vi "getSerializedData.vi"(0 "reference":refnum<class "InterfaceNode.lvclass">, 5 "error in (no error)":errorcluster) -> (14 "reference out":refnum<class "InterfaceNode.lvclass">, 15 "parent":refnum<class "AbstractNode.lvclass">, 16 "children":refnum<class "AbstractNode.lvclass">[](array[class]), 17 "xmlOut":string, 19 "error out":errorcluster)   [LabVIEW 2020, in "InterfaceNode.lvclass"]
doc: "getSerializedData"
uses:
  <resource>/Framework/Providers/Open_GDS/UML/InterfaceNode_class/InterfaceNode.lvclass
  C:/Program Files (x86)/National Instruments/LabVIEW 2020/resource/Framework/Providers/Open_GDS/UML/ClassNode_class/ClassNode.lvclass
  C:/Program Files (x86)/National Instruments/LabVIEW 2020/resource/Framework/Providers/Open_GDS/UML/RectangularNode_class/RectangularNode.lvclass
  C:/Program Files (x86)/National Instruments/LabVIEW 2020/resource/Framework/Providers/Open_GDS/UML/AbstractNode_class/AbstractNode.lvclass
  <resource>/Framework/Providers/Open_GDS/UML/AbstractNode_class/AbstractNode.lvclass
  <resource>/Framework/Providers/Open_GDS/UML/General/Rectangle/Rectangle Rectangle2D.ctl
  <resource>/Framework/Providers/Open_GDS/UML/MultiLineString_class/MultiLineString.lvclass
  <resource>/Framework/Providers/Open_GDS/UML/ClassNode_class/ClassNode.lvclass
  <resource>/Framework/Providers/Open_GDS/UML/RectangularNode_class/RectangularNode.lvclass
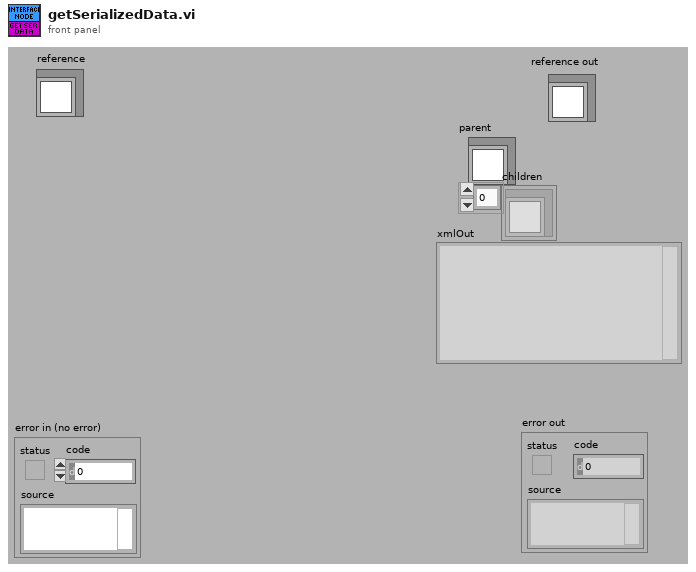
[diagram p1: front panel]
types:
  T1 = typedef "Rectangle Rectangle2D.ctl" = cluster{"x":dbl, "y":dbl, "width":dbl, "height":dbl}
  T2 = cluster{"Base class":cluster{"Base class":cluster{"parent":refnum<k1>, "children":refnum<k1>[], "Hidden":bool}, "bounds":T1}, "midHeight":dbl, "botHeight":dbl, "name":refnum<k1>, "attributes":refnum<k1>, "methods":refnum<k1>, "DEFAULT_COMPARTMENT_HEIGHT":i32, "DEFAULT_WIDTH":i32, "DEFAULT_HEIGHT":i32, "showMethods":bool, "showAttributes":bool, "ClassPath":path}
  T3 = typedef "ClassNode.lvclass/ObjectAttributes.ctl" = cluster{"midHeight":dbl, "botHeight":dbl, "name":refnum<class "MultiLineString.lvclass">, "attributes":refnum<class "MultiLineString.lvclass">, "methods":refnum<class "MultiLineString.lvclass">, "DEFAULT_COMPARTMENT_HEIGHT":i32, "DEFAULT_WIDTH":i32, "DEFAULT_HEIGHT":i32, "showMethods":bool, "showAttributes":bool, "ClassPath":path}
  T4 = typedef "RectangularNode.lvclass/ObjectAttributes.ctl" = cluster{"bounds":T1}
  T5 = typedef "AbstractNode.lvclass/ObjectAttributes.ctl" = cluster{"parent":refnum<class "AbstractNode.lvclass">, "children":refnum<class "AbstractNode.lvclass">[], "Hidden":bool}
  T6 = cluster{"Attributes":cluster{"Base class":cluster{"Base class":cluster{"parent":refnum<k1>, "children":refnum<k1>[], "Hidden":bool}, "bounds":T1}, "midHeight":dbl, "botHeight":dbl, "name":refnum<k1>, "attributes":refnum<k1>, "methods":refnum<k1>, "DEFAULT_COMPARTMENT_HEIGHT":i32, "DEFAULT_WIDTH":i32, "DEFAULT_HEIGHT":i32, "showMethods":bool, "showAttributes":bool, "ClassPath":path}, "text":string, "text":string}
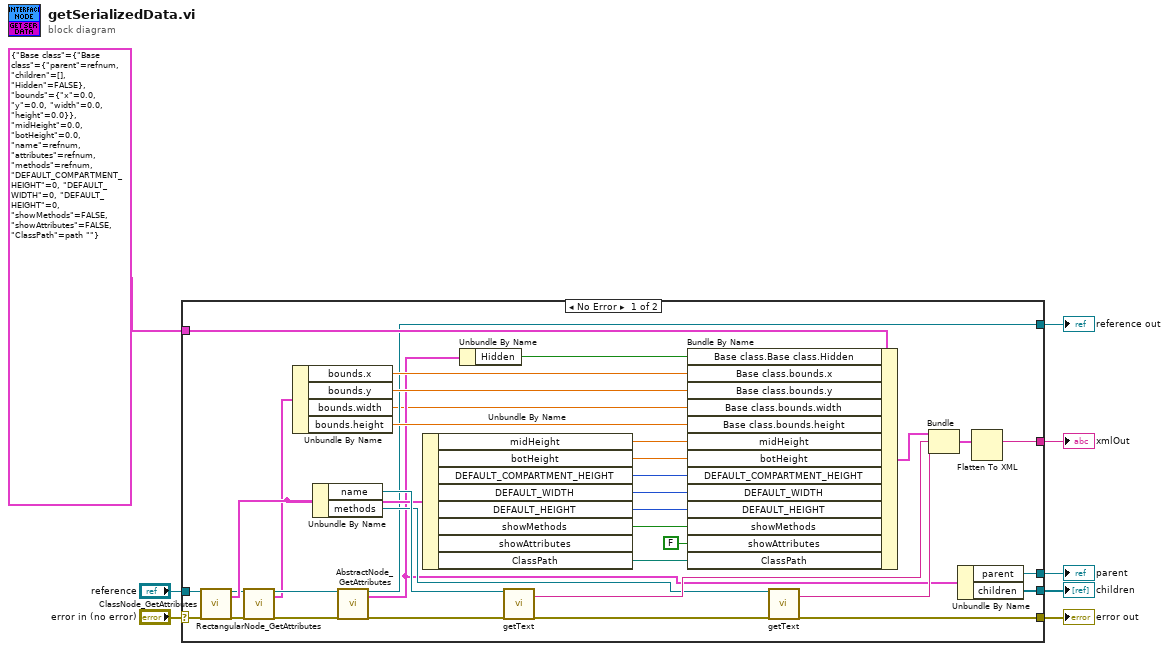
[diagram p0: block diagram]
diagram:
  n1 = case shown="No Error" "error in (no error)" {
    selector: "error in (no error)" -> [w44 w45]
    tunnel: "reference" -> [w43 w46]
    tunnel: [w36 w45] -> w6
    tunnel: [w15 w46] -> w5
    tunnel: [w35 _] -> w4
    tunnel: [w34 _] -> w3
    tunnel: [w33 _] -> w2
    tunnel: T2 {"Base class"={"Base class"={"parent"=refnum, "children"=[], "Hidden"=FALSE}, "bounds"={"x"=0.0, "y"=0.0, "width"=0.0, "height"=0.0}}, "midHeight"=0.0, "botHeight"=0.0, "name"=refnum, "attributes"=refnum, "methods"=refnum, "DEFAULT_COMPARTMENT_HEIGHT"=0, "DEFAULT_WIDTH"=0, "DEFAULT_HEIGHT"=0, "showMethods"=FALSE, "showAttributes"=FALSE, "ClassPath"=path ""} ("Attributes") -> [w24 _]
    frame No Error {
      n2 = call <resource>:"ClassNode_GetAttributes.vi"("reference in"=w43, "error in (no error)"=w44) -> ("reference out"=w20:refnum<class "InterfaceNode.lvclass">, "Data"=w21:T3, "error out"=w19:errorcluster)  [unwired: 14 in, 1 out]
      n3 = call <resource>:"RectangularNode_GetAttributes.vi"("reference in"=w20, "error in (no error)"=w19) -> ("reference out"=w18:refnum<class "InterfaceNode.lvclass">, "Data"=w13:T4, "error out"=w17:errorcluster)  [unwired: 14 in, 1 out]
      n4 = Unbundle By Name(w13) -> ("bounds.x"=w32:dbl, "bounds.y"=w31:dbl, "bounds.width"=w12:dbl, "bounds.height"=w30:dbl)
      n5 = Unbundle By Name(w21) -> ("name"=w41:refnum<class "MultiLineString.lvclass">, "methods"=w38:refnum<class "MultiLineString.lvclass">)
      n6 = call <resource>:"AbstractNode_GetAttributes.vi"("reference in"=w18, "error in (no error)"=w17) -> ("reference out"=w15:refnum<class "InterfaceNode.lvclass">, "Data"=w14:T5, "error out"=w16:errorcluster)  [unwired: 14 in, 1 out]
      n7 = Unbundle By Name(w21) -> ("midHeight"=w28:dbl, "botHeight"=w29:dbl, "DEFAULT_COMPARTMENT_HEIGHT"=w27:i32, "DEFAULT_WIDTH"=w26:i32, "DEFAULT_HEIGHT"=w25:i32, "showMethods"=w10:bool, "ClassPath"=w11:path)  [unwired: 1 out]
      n8 = Unbundle By Name(w14) -> ("Hidden"=w22:bool)
      n9 = call-dynamic "getText.vi"("reference"=w41, "error in (no error)"=w16) -> ("text"=w40:string, "error out"=w37:errorcluster)  [unwired: 16 out]
      n10 = Bundle By Name(cluster=w24, "Base class.Base class.Hidden"=w22, "Base class.bounds.x"=w32, "Base class.bounds.y"=w31, "Base class.bounds.width"=w12, "Base class.bounds.height"=w30, "midHeight"=w28, "botHeight"=w29, "DEFAULT_COMPARTMENT_HEIGHT"=w27, "DEFAULT_WIDTH"=w26, "DEFAULT_HEIGHT"=w25, "showMethods"=w10, "showAttributes"=FALSE, "ClassPath"=w11) -> (w23:T2)
      n11 = call-dynamic "getText.vi"("reference"=w38, "error in (no error)"=w37) -> ("text"=w39:string, "error out"=w36:errorcluster)  [unwired: 16 out]
      n12 = Bundle("Attributes"=w23, "text"=w40, "text"=w39) -> (w42:T6)  [unwired: 1 out]
      n13 = Unbundle By Name(w14) -> ("parent"=w35:refnum<class "AbstractNode.lvclass">, "children"=w34:refnum<class "AbstractNode.lvclass">[])
      n14 = Flatten To XML(6:w42) -> (2:w33:string)
    }
    frame Error {
    }
  }
  "reference out" <- w5
  "error out" <- w6
  "parent" <- w4
  "children" <- w3
  "xmlOut" <- w2
